vi "VIH Project Tree - Create Unique Output Names for Added Files.vi"(8 "error in":errorcluster, 9 "Check All (F)":bool, 10 "Added Item Tags":string[](array[string]), 11 "Project Tree":T1) -> (0 "error out":errorcluster, 3 "dup Project Tree":T1)   [LabVIEW 2014]
doc: "::: VI Helpeks :::\nCopyright (c) 2000-2026 Konstantin Shifershteyn. All rights reserved."
uses:
  VIH Project Tree Typedef - Tree Refnum.ctl
  _VIH HelpGen - Palette.llb/VIH HelpGen Typedef - Palette - Item Type Enum.ctl
panel:
  # "VI Helpeks\nCopyright (c) 2012-2026 Konstantin Shifershteyn"
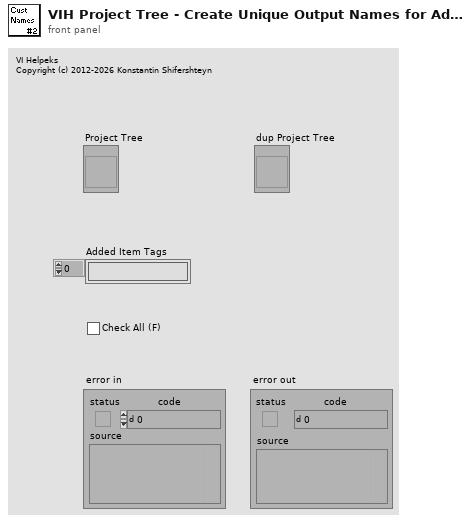
[diagram p1: front panel]
types:
  T1 = typedef "VIH Project Tree Typedef - Tree Refnum.ctl" = refnum<vi>
  T2 = typedef "VIH HelpGen Typedef - Palette - Item Type Enum.ctl" = enum32{"<Invalid>", "<unknown>", "VI", "Menu", "LV Func", "Express VI", "Poly VI", "CTL", "HTML"}
  T3 = typedef "VIH Project Tree Typedef - Tree Item Type.ctl" = enum32{"<Invalid>", "Project", "Proj Files", "Proj Rules", "File Group", "Rule Group", "Any File", "LV Func", ".mnu", ".mnu (dyn)", ".vi", ".vi (dyn)", ".vit", ".vit (dyn)", ".ctl", ".ctl (dyn)", ".ctt", ".ctt (dyn)", "polyVI", "polyVI (dyn)", "expVI", "expVI (dyn)", "HTML", "PolyVI Inst"}
  T4 = typedef "VIH HelpGen Typedef - Cluster - File Rule.ctl" = cluster{"OutName":string, "BuildHelp":T5, "Source Paths":T6, "Target Paths":T7, "DscrMode":T8, "Description":string, "Control Rules":T9[], "Flags":T11, "Ctl_DscrMode":T8, "Ctl_ClustMembers":T5, "Ctl_EnumValues":T5, "MenuItemIcons":T5, "%Comments":string, "DetailsMode":T8, "DetailsText":string, "ProductInfoMode":T5, "ProductInfoText":string}
  T5 = typedef "VIH HelpGen Typedef - Enum - Default,Enable,Disable.ctl" = enum16{"Default", "Enable", "Disable"}
  T6 = typedef "VIH HelpGen Typedef - Cluster - File Rule - Source Paths.ctl" = cluster{"CSS Files":path[], "JS Files":path[], "Html Template":path}
  T7 = typedef "VIH HelpGen Typedef - Cluster - File Rule - Target Paths.ctl" = cluster{"HTML Dir":path, "Image Dir":path, "CSS Dir":path, "JS Dir":path}
  T8 = typedef "VIH HelpGen Typedef - Enum - Description Mode.ctl" = enum16{"Default", "Description", "Description1", "Description2", "Custom", "None"}
  T9 = typedef "VIH HelpGen Typedef - Cluster - Control Rule.ctl" = cluster{"CtrlID":string, "CustomRule":bool, "DscrMode":T8, "Description":string, "ClusterMembers":T5, "EnumValues":T5, "EnumValDscr":T10[], "CustomName":string}
  T10 = typedef "VIH HelpGen Typedef - Cluster - Enum Value Info.ctl" = cluster{"Value":ext, "String":string, "Description":string}
  T11 = typedef "VIH HelpGen Typedef - Cluster - Group Rule - Flags.ctl" = cluster{"Override CSS Files":bool, "Override JS Files":bool, "Override Ctl Rules":bool}
  T12 = enum16{"get", "get all", "set", "Init", "delete", "rename"}
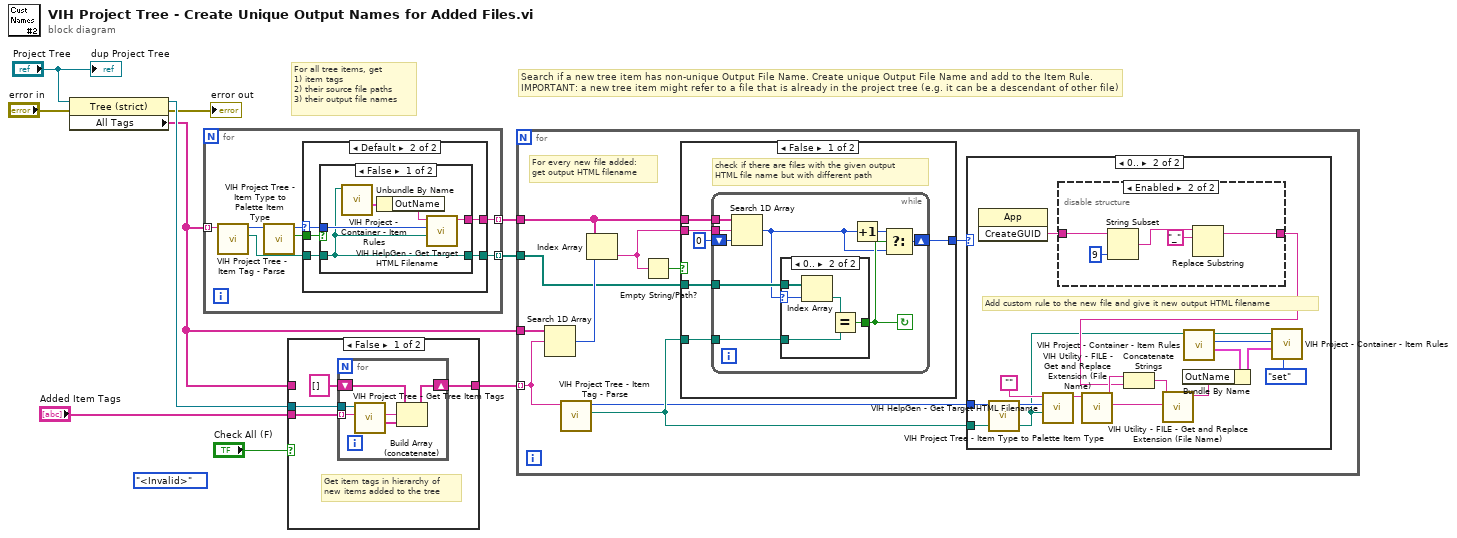
[diagram p0: block diagram]
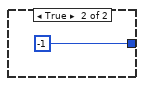
[diagram p4: hidden frame]
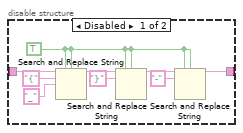
[diagram p6: hidden frame]
diagram:
  (unwired) VIH_HelpGen_Typedef_-_Palette_-_Item_Type_Enum."<Invalid>" ("Item/File Type")
  # "Search if a new tree item has non-unique Output File Name. Create unique Output File Name and add to the Item Rule.\nIMPORTANT: a new tree item might refer to a file that is already in the project tree (e.g. it can be a descendant of other file)"
  # "For all tree items, get \n1) item tags\n2) their source file paths \n3) their output file names"
  n1 = property class="Tree (strict)"(reference="Project Tree", error in="error in") -> (reference out=w8:T1, error out=→"error out":errorcluster, "All Tags"=w1:string[])
  n2 = for {
    tunnel: w1 -> [w17] mode=indexing
    tunnel: [w14] -> w3 mode=indexing
    tunnel: [w11] -> w4 mode=indexing
    n3 = call "VIH Project Tree - Item Tag - Parse.vi"("Tree Item Tag"=w17) -> ("Item File Path"=w15:path, "Item Type"=w16:T3)  [unwired: 8 in, 1 out]
    n4 = call "VIH Project Tree - Item Type to Palette Item Type.vi"("Tree Item Type"=w16) -> ("PolyVI Instance VI"=w12:bool, "Item/File Type"=w13:T2)  [unwired: 9 in]
    n5 = case shown="Default" w13 {
      selector: w13 -> [_ w20]
      tunnel: w15 -> [_ w22]
      tunnel: [_ w21] -> w14
      tunnel: w12 -> [_ w19]
      tunnel: [_ w18] -> w11
      frame "<Invalid>" {
      }
      frame Default {
        n6 = case shown="False" w19 {
          tunnel: w22 -> [w23 _]
          tunnel: [w25 _] -> w21
          tunnel: w20 -> [w24 _]
          tunnel: [w23 _] -> w18
          frame False {
            n7 = call "VIH Project - Container - Item Rules.vi"("Item Path"=w23) -> ("Item Rule out"=w26:T4)  [unwired: 6 in, 4 out]
            n8 = Unbundle By Name(w26) -> ("OutName"=w27:string)
            n9 = call "VIH HelpGen - Get Target HTML Filename.vi"("Item File Path"=w23, "Item Type"=w24, "HTML Filename in"=w27) -> ("HTML Fileame out"=w25:string)  [unwired: 7 in, 1 out]
          }
          frame True {
          }
        }
      }
    }
  }
  n10 = case shown="False" "Check All (F)" {
    tunnel: "Added Item Tags" -> [w31 _]
    tunnel: w8 -> [w29 _]
    tunnel: [w28 w38] -> w5
    tunnel: w1 -> [_ w38]
    frame False {
      # "Get item tags in hierarchy of\nnew items added to the tree"
      n11 = for {
        tunnel: w29 -> [w37]
        tunnel: w31 -> [w36] mode=indexing
        shift-right: [w32] -> w28
        shift-left: string[] [] -> [w33]
        n12 = call "VIH Project Tree - Get Tree Item Tags.vi"("Parent Item Tag"=w36, "Project Tree"=w37) -> ("Child Item Tags"=w34:string[], "dup Parent Item Tag"=w35:string)  [unwired: 6 in, 2 out]
        n13 = Build Array (concatenate)(w33, w35, w34) -> (w32:string[])
      }
    }
    frame True {
    }
  }
  n14 = for {
    tunnel: w5 -> [w43] mode=indexing
    tunnel: w1 -> [w48]
    tunnel: w4 -> [w45]
    tunnel: w3 -> [w46]
    # "For every new file added:\nget output HTML filename"
    n15 = Search 1D Array(1D array=w48, element=w43) -> (index of element=w47:i32)  [unwired: 1 in]
    n16 = call "VIH Project Tree - Item Tag - Parse.vi"("Tree Item Tag"=w43) -> ("Item File Path"=w42:path, "Item Type"=w41:T3)  [unwired: 8 in, 1 out]
    n17 = Index Array(array=w46, index=w47) -> (element=w40:string)
    n18 = Empty String/Path?(string/path=w40) -> (empty?=w39:bool)
    n19 = case shown="False" w39 {
      tunnel: w46 -> [w54 _]
      tunnel: w45 -> [w52 _]
      tunnel: [w51 -1 ("index of element")] -> w44
      tunnel: w42 -> [w50 _]
      tunnel: w40 -> [w49 _]
      frame False {
        # "check if there are files with the given output\nHTML file name but with different path"
        n20 = while {
          tunnel: w54 -> [w63]
          tunnel: w49 -> [w62]
          shift-right: [w57] -> w51
          shift-left: 0 ("index of element") -> [w61]
          tunnel: w52 -> [w60]
          tunnel: w50 -> [w59]
          stop <- w58 continue-if-true
          n21 = Search 1D Array(1D array=w63, element=w62, start index (0)=w61) -> (index of element=w55:i32)
          n22 = case shown="0.." w55 {
            selector: w55 -> [_ w68]
            tunnel: w60 -> [_ w67]
            tunnel: w59 -> [_ w65]
            tunnel: [_ w64] -> w58
            frame ..-1 {
            }
            frame 0.. {
              n23 = Index Array(array=w67, index=w68) -> (element=w66:path)
              n24 = Equal?(x=w66, y=w65) -> (x = y?=w64:bool)
            }
          }
          n25 = Increment(x=w55) -> (x+1=w56:i32)
          n26 = Select(t=w56, s=w58, f=w55) -> (s? t:f=w57:i32)
        }
      }
      frame True {
      }
    }
    n27 = case shown="0.." w44 {
      tunnel: w42 -> [_ w70]
      tunnel: w41 -> [_ w71]
      frame ..-1 {
      }
      frame 0.. {
        # "Add custom rule to the new file and give it new output HTML filename"
        n28 = invoke class="App" method="CreateGUID"() -> ("CreateGUID"=w74:string)  [unwired: 3 in, 2 out]
        n29 = call "VIH Project Tree - Item Type to Palette Item Type.vi"("Tree Item Type"=w71) -> ("Item/File Type"=w80:T2)  [unwired: 9 in, 1 out]
        n30 = call "VIH HelpGen - Get Target HTML Filename.vi"("Item File Path"=w70, "Item Type"=w80, "HTML Filename in"="") -> ("HTML Fileame out"=w79:string)  [unwired: 7 in, 1 out]
        n31 = disable-structure shown="Enabled" {
          disable-tunnel: w74 -> [w94 w97]
          disable-tunnel: [w86 w95] -> w73
          frame Disabled {
            w87 = TRUE
            n32 = Search and Replace String(replace all?=w87, case sensitive?=w87, input string=w94, search string="{", replace string="_" ("replace string (\"\")")) -> (result string=w91:string)  [unwired: 3 in, 3 out]
            n33 = Search and Replace String(replace all?=w87, case sensitive?=w87, input string=w91, search string="}") -> (result string=w90:string)  [unwired: 4 in, 3 out]
            n34 = Search and Replace String(replace all?=w87, case sensitive?=w87, input string=w90, search string="-") -> (result string=w86:string)  [unwired: 4 in, 3 out]
          }
          frame Enabled {
            n35 = String Subset(string=w97, length (rest)=9 ("length (rest)")) -> (substring=w96:string)  [unwired: 1 in]
            n36 = Replace Substring(4:"_" ("substring (\"\")"), 5:w96) -> (1:w95:string)  [unwired: 2 in, 1 out]
          }
        }
        n37 = call "VIH Utility - FILE - Get and Replace Extension (File Name).vi"("File name"=w79) -> ("extension"=w77:string, "File name out"=w78:string)  [unwired: 9 in]
        n38 = Concatenate Strings(w78, w73) -> (w76:string)
        n39 = call "VIH Utility - FILE - Get and Replace Extension (File Name).vi"("new extension (none)"=w77, "File name"=w76) -> ("File name out"=w75:string)  [unwired: 8 in, 1 out]
        n40 = call "VIH Project - Container - Item Rules.vi"("Item Path"=w70) -> ("Item Rule out"=w83:T4, "Item Idx out"=w85:i32, "Item Path out"=w84:path)  [unwired: 6 in, 2 out]
        n41 = Bundle By Name(cluster=w83, "OutName"=w75) -> (w82:T4)
        n42 = call "VIH Project - Container - Item Rules.vi"("cmd (get)"=T12."set", "Item Rule"=w82, "Item Idx (-1)"=w85, "Item Path"=w84) -> ()  [unwired: 3 in, 5 out]
      }
    }
  }
  "dup Project Tree" <- "Project Tree"
